vi "Create SimpleText Paragraph.vi"(8 "error in (no error)":errorcluster, 10 "simpleText":string, 11 "ooCalc in":refnum<class "ooCalc.lvclass">) -> (0 "error out":errorcluster, 2 "SimpleTextParagraph":refnum<k24>, 3 "ooCalc out":refnum<class "ooCalc.lvclass">)   [LabVIEW 2009, in "ooCalc.lvclass"]
uses:
  ooCalc.lvclass
  C:/Projets/LAVAG/OpenOfficeRGT/AODL/DLLs/AODL.dll
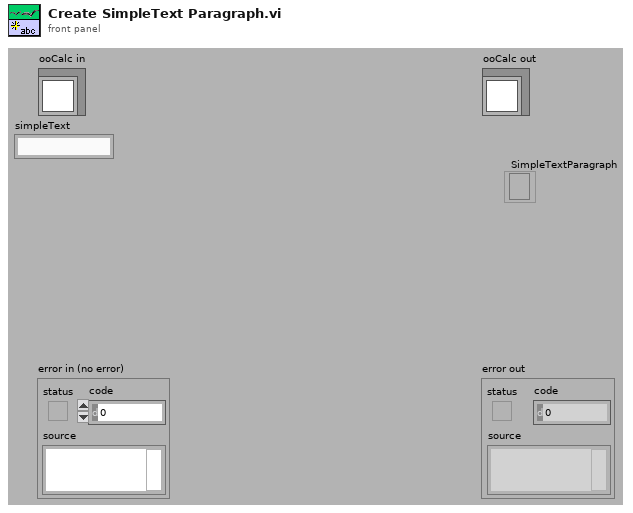
[diagram p1: front panel]
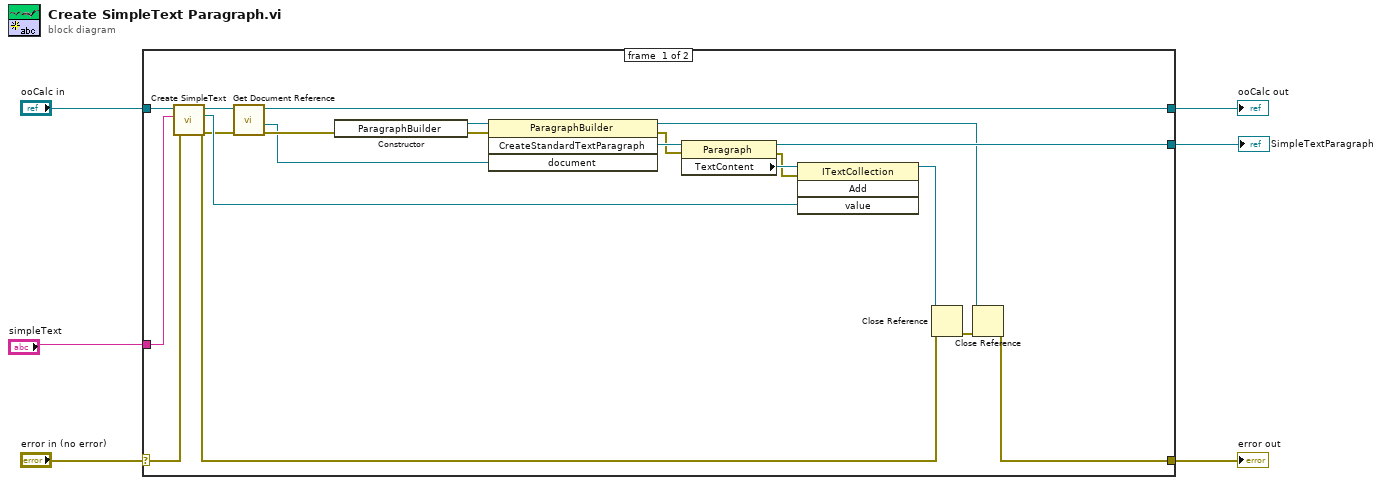
[diagram p0: block diagram]
diagram:
  n1 = case shown="No Error" "error in (no error)" {
    selector: "error in (no error)" -> [w21 w28]
    tunnel: [w12 w28] -> w5
    tunnel: [w10 w27] -> w3
    tunnel: "ooCalc in" -> [w22 w27]
    tunnel: "simpleText" -> [w19 _]
    tunnel: [w23 _] -> w1
    frame #0 {
      n2 = call-dynamic "Create SimpleText.vi"("error in (no error)"=w21, "simpleText"=w19, "ooDocument"=w22) -> ("error out"=w9:errorcluster, "SimpleText"=w20:refnum<k24>, "ooDocument out"=w11:refnum<class "ooCalc.lvclass">)  [unwired: 6 in]
      n3 = call-dynamic "Get Document Reference.vi"("error in (no error)"=w9, "ooDocument in"=w11) -> ("error out"=w8:errorcluster, "Document"=w7:refnum<k24>, "ooDocument out"=w10:refnum<class "ooCalc.lvclass">)  [unwired: 7 in]
      n4 = constructor class="ParagraphBuilder"(error in=w8) -> (reference out=w25:refnum<k24>, error out=w26:errorcluster)  [unwired: 2 in, 1 out]
      n5 = invoke class="ParagraphBuilder" method="CreateStandardTextParagraph"(reference=w25, error in=w26, "document"=w7) -> (reference out=w13:refnum<k24>, error out=w16:errorcluster, "CreateStandardTextParagraph"=w17:refnum<k24>)  [unwired: 1 in, 1 out]
      n6 = property class="Paragraph"(reference=w17, error in=w16) -> (reference out=w23:refnum<k24>, error out=w15:errorcluster, "TextContent"=w24:refnum<k24>)
      n7 = invoke class="ITextCollection" method="Add"(reference=w24, error in=w15, "value"=w20) -> (reference out=w14:refnum<k24>)  [unwired: 1 in, 3 out]
      n8 = Close Reference(reference=w14, error in (no error)=w9) -> (error out=w18:errorcluster)
      n9 = Close Reference(reference=w13, error in (no error)=w18) -> (error out=w12:errorcluster)
    }
    frame #1 {
    }
  }
  "error out" <- w5
  "ooCalc out" <- w3
  "SimpleTextParagraph" <- w1
